vi "Config_Get_Active.vi"(8 "error in (no error)":errorcluster={"status"=FALSE, "code"=0, "source"="\"\""}, 10 "requested ID":string, 11 "Snapshot handle":string) -> (0 "error out":errorcluster={"status"=FALSE, "code"=0, "source"="\"\""}, 2 "status ok":bool, 3 "Typed definition/result":string)   [LabVIEW 2026]
doc: "INTENT: Return read-only run configuration. LOGIC: Retrieve by identifier without exposing writeable storage."
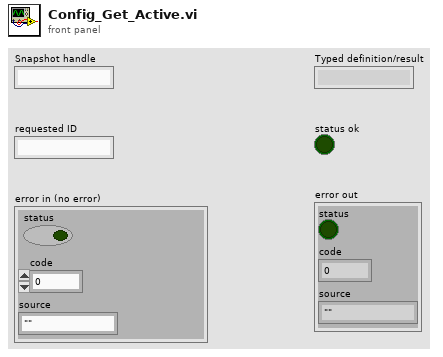
[diagram p1: front panel]
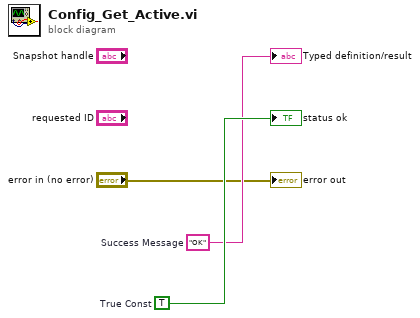
[diagram p0: block diagram]
diagram:
  w3 = TRUE  # True Const
  w2 = "OK"  # Success Message
  "Typed definition/result" <- w2
  "status ok" <- w3
  "error out" <- "error in (no error)"
